vi "Image Acquisition.vi"() -> ()   [LabVIEW 2025]
uses:
  VIs_needed/Grab Manager Mode.ctl
  <vilib>/vision/driver/IMAQdx.llb/IMAQdx Buffer Number Mode.ctl
  <vilib>/Utility/High Resolution Relative Seconds.vi
  <vilib>/vision/driver/NI_Vision_Acquisition_Software.lvlib
  <resource>/objmgr/imaqdx.rc
panel:
  out "Times between Frames":u32
  in  "Output Folder":path
  in  "Stop":bool
  out "Images Saved Per Second":dbl
  out "Images Behind":i32
  out "Images Acquired Per Second":dbl
  in  "Skip Count":u32
  out "Write Speed Waveform":dbl(graph) caption="Image File Write Speed"
  in  "Number of Images":u32=30
  in  "Camera Name":refnum<k21> caption="IMAQdx Session"
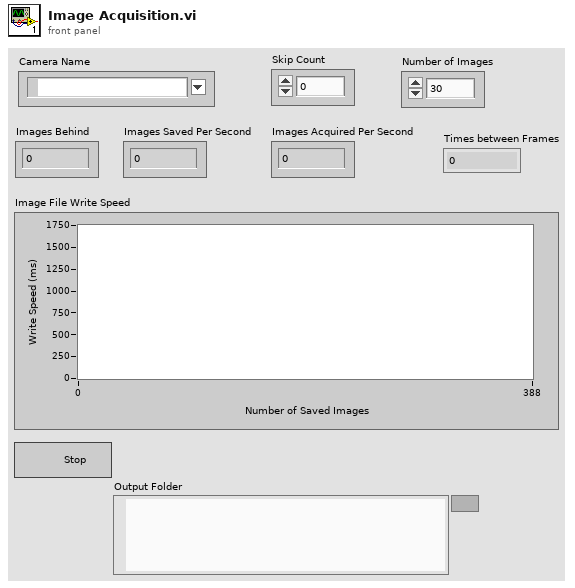
[diagram p1: front panel]
types:
  T1 = typedef "Grab Manager Mode.ctl" = enum16{"Create Processing Images", "Lock", "Add Acquired Image", "Get Acquired Image", "Unlock", "Dispose Processing Images"}
  T2 = cluster{"Number of Processing Images":u32, "Image Border Size":u32}
  T3 = typedef "IMAQdx.ctl" = refnum<k21>
  T4 = typedef "NI_Vision_Acquisition_Software.lvlib/IMAQdx Buffer Number Mode.ctl" = enum32{"Next", "Last", "Buffer Number", "Every", "Last New"}
  T5 = typedef "IMAQ Image.ctl" = refnum<image>
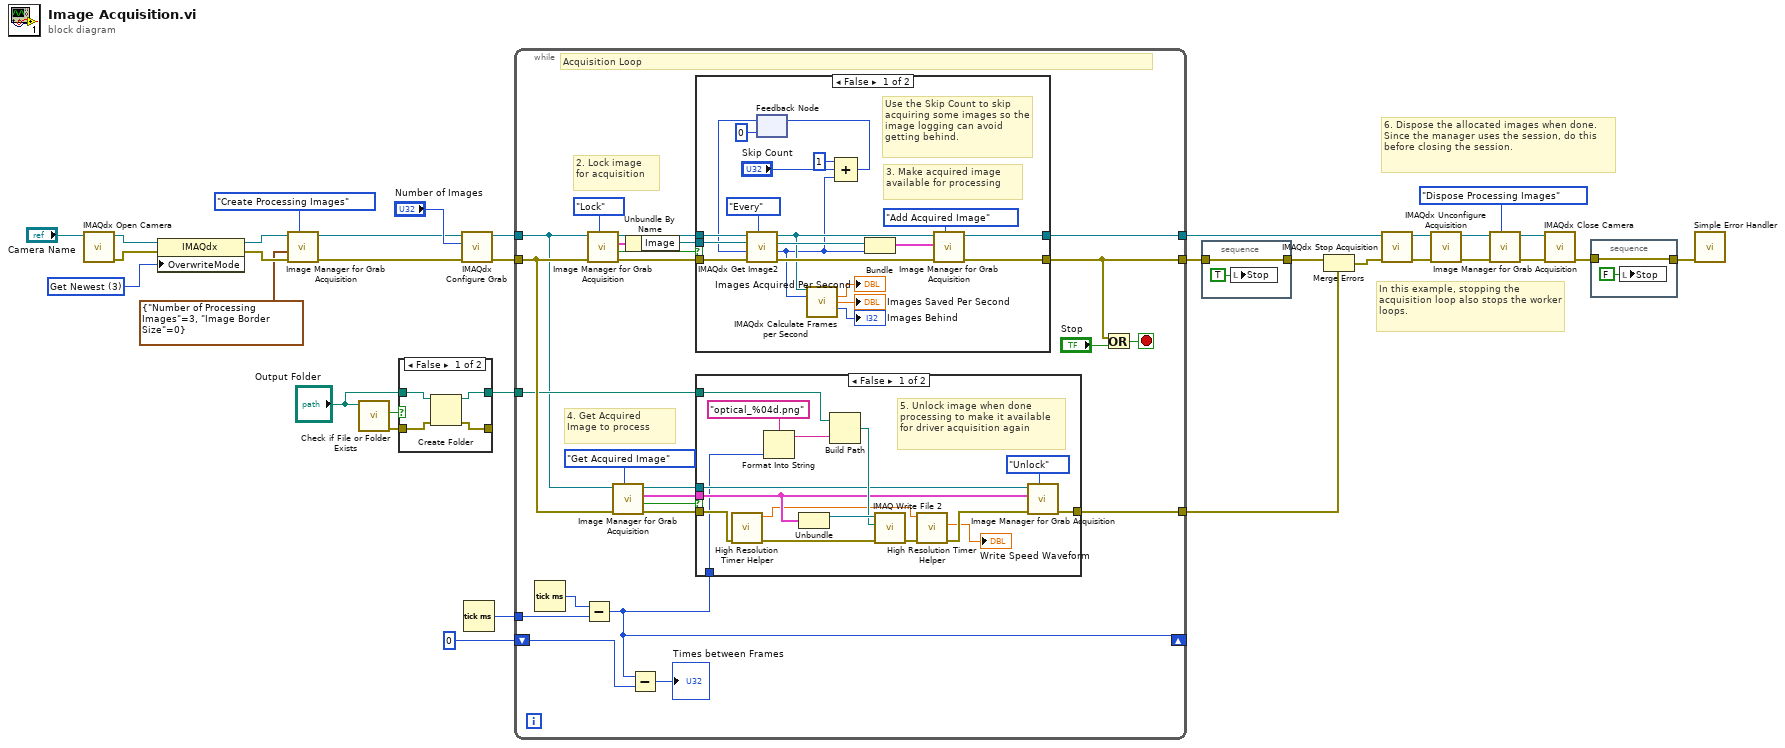
[diagram p0: block diagram]
diagram:
  w32 = u32 3 items=["Get Oldest"=0, "Fail"=2, "Get Newest"=3] ("OverwriteMode")
  # "6. Dispose the allocated images when done. Since the manager uses the session, do this before closing the session."
  # "In this example, stopping the acquisition loop also stops the worker loops."
  n1 = call <vilib>:"IMAQdx Open Camera.vi"("Session In"="Camera Name") -> ("error out"=w28:errorcluster, "Session Out"=w29:T3)  [unwired: 2 in, 7 out]
  n2 = property class="IMAQdx"(reference=w29, error in=w28, "OverwriteMode"=w32) -> (reference out=w31:T3, error out=w30:errorcluster)
  n3 = call "Image Manager for Grab Acquisition.vi"("Mode"=Grab_Manager_Mode."Create Processing Images", "error in (no error)"=w30, "Init Settings"=T2 {"Number of Processing Images"=3, "Image Border Size"=0}, "Session In"=w31) -> ("error out"=w24:errorcluster, "Session Out"=w23:T3)  [unwired: 4 in, 2 out]
  n4 = call <vilib>:"Check if File or Folder Exists.vi"("path"="Output Folder") -> ("error out"=w4:errorcluster, "file or folder exists?"=w6:bool)  [unwired: 8 in, 1 out]
  n5 = case shown="False" w6 {
    tunnel: "Output Folder" -> [w37 w39]
    tunnel: [w36 w39] -> w3
    tunnel: w4 -> [w35 w38]
    tunnel: [w34 w38] -> _
    frame False {
      n6 = Create Folder(path (use dialog)=w37, error in=w35) -> (created path=w36:path, error out=w34:errorcluster)  [unwired: 1 in, 1 out]
    }
    frame True {
    }
  }
  n7 = call <vilib>:"IMAQdx Configure Grab.vi"("error in"=w24, "Number of Buffers"="Number of Images", "Session In"=w23) -> ("error out"=w7:errorcluster, "Session Out"=w8:T3)  [unwired: 7 in]
  n8 = Tick Count (ms)() -> (millisecond timer value=w2:u32)
  n9 = while {
    tunnel: w7 -> [w53]
    tunnel: w8 -> [w51]
    tunnel: [w60] -> w19
    tunnel: [w61] -> w18
    tunnel: w3 -> [w52]
    tunnel: [w50] -> w9
    tunnel: w2 -> [w43]
    shift-right: [w40] -> _
    shift-left: u32 0 -> [w41]
    stop <- w62 stop-if-true
    # "4. Get Acquired Image to process"
    # "2. Lock image for acquisition"
    # "Acquisition Loop"
    n10 = Tick Count (ms)() -> (millisecond timer value=w44:u32)
    n11 = Subtract(x=w44, y=w43) -> (x-y=w40:u32)
    n12 = call "Image Manager for Grab Acquisition.vi"("Mode"=Grab_Manager_Mode."Lock", "error in (no error)"=w53, "Session In"=w51) -> ("error out"=w56:errorcluster, "No Available Image"=w57:bool, "Image Settings Out"=w55:cluster{"Image":T5, "Buffer Number":u32}, "Session Out"=w58:T3)  [unwired: 5 in]
    n13 = call "Image Manager for Grab Acquisition.vi"("Mode"=Grab_Manager_Mode."Get Acquired Image", "error in (no error)"=w53, "Session In"=w51) -> ("error out"=w46:errorcluster, "No Available Image"=w48:bool, "Image Settings Out"=w47:cluster{"Image":T5, "Buffer Number":u32}, "Session Out"=w45:T3)  [unwired: 5 in]
    n14 = Unbundle By Name(w55) -> ("Image"=w54:T5)
    n15 = Subtract(x=w40, y=w41) -> (x-y=→"Times between Frames":u32)
    n16 = case shown="False" w57 {
      tunnel: [w92 w102] -> w60
      tunnel: [w91 w101] -> w61
      tunnel: w58 -> [w100 w102]
      tunnel: w56 -> [w99 w101]
      tunnel: w54 -> [w93 _]
      frame False {
        # "3. Make acquired image available for processing"
        # "Use the Skip Count to skip acquiring some images so the image logging can avoid getting behind."
        n17 = feedback #1(u32 0) -> (w82:u32)
        n18 = call <vilib>:"IMAQdx Get Image2.vi"("Buffer Number Mode (Next)"=IMAQdx_Buffer_Number_Mode."Every", "error in"=w99, "Buffer Number In"=w82, "Image In"=w93, "Session In"=w100) -> ("error out"=w95:errorcluster, "Buffer Number Out"=w86:u32, "Image Out"=w97:T5, "Session Out"=w90:T3)  [unwired: 3 in]
        n19 = call <vilib>:"IMAQdx Calculate Frames per Second.vi"("Session In"=w90, "Buffer Number"=w86) -> ("Acquired Frames per Second"=→"Images Acquired Per Second":dbl, "Processed Frames per Second"=→"Images Saved Per Second":dbl, "Images Behind"=→"Images Behind":i32)  [unwired: 7 in, 4 out]
        n20 = Compound Arithmetic op=ADD(u32 1 ("value"), "Skip Count", w86) -> (w83:u32)
        n21 = feedback-in #1(w83) -> ()
        n22 = Bundle("Image Out"=w97, "Buffer Number Out"=w86) -> (w96:cluster{"Image Out":T5, "Buffer Number Out":u32})  [unwired: 1 in]
        n23 = call "Image Manager for Grab Acquisition.vi"("Mode"=Grab_Manager_Mode."Add Acquired Image", "error in (no error)"=w95, "Image Settings In"=w96, "Session In"=w90) -> ("error out"=w91:errorcluster, "Session Out"=w92:T3)  [unwired: 4 in, 2 out]
      }
      frame True {
        # "The Lock function already has a delay inside when no images are available to prevent loop from going too fast and starving the worker threads from getting processing time."
        # "Write to disk operation is taking longer so images aren't added back to manager. Wait until there is an available image"
      }
    }
    n24 = case shown="False" w48 {
      tunnel: w46 -> [w70 w80]
      tunnel: w47 -> [w72 _]
      tunnel: [w74 w80] -> w50
      tunnel: w52 -> [w78 _]
      tunnel: w45 -> [w71 _]
      tunnel: w40 -> [w64 _]
      frame False {
        # "5. Unlock image when done processing to make it available for driver acquisition again"
        n25 = call "High Resolution Timer Helper.vi"("error in (no error)"=w70) -> ("error out"=w69:errorcluster, "Current Time"=w65:dbl)  [unwired: 8 in, 1 out]
        n26 = Format Into String(format string="optical_%04d.png", w64) -> (resulting string=w77:string)  [unwired: 2 in, 1 out]
        n27 = Unbundle(w72) -> ("Image"=w79:T5)  [unwired: 1 out]
        n28 = Build Path(base path=w78, name or relative path=w77) -> (appended path=w75:path)
        n29 = call-poly "IMAQ Write File 2"("error in (no error)"=w69, "File Path"=w75, "Image"=w79) -> ("error out"=w68:errorcluster)  [unwired: 7 in, 1 out]
        n30 = call "High Resolution Timer Helper.vi"("error in (no error)"=w68, "Previous Time"=w65) -> ("error out"=w67:errorcluster, "Time Difference (ms)"=→"Write Speed Waveform":dbl)  [unwired: 7 in, 1 out]
        n31 = call "Image Manager for Grab Acquisition.vi"("Mode"=Grab_Manager_Mode."Unlock", "error in (no error)"=w67, "Image Settings In"=w72, "Session In"=w71) -> ("error out"=w74:errorcluster)  [unwired: 4 in, 3 out]
      }
      frame True {
        # "No acquired images to process"
      }
    }
    n32 = Or(x=w61, y="Stop") -> (x .or. y?=w62:bool)
  }
  n33 = stacked-sequence {
    tunnel: [w103] -> w17
    tunnel: w18 -> [w103]
    frame #0 {
      n34 = local write "Stop"(TRUE ("Stop")) -> ()
    }
  }
  n35 = Merge Errors(w17, w9) -> (w20:errorcluster)
  n36 = call <vilib>:"IMAQdx Stop Acquisition.vi"("error in"=w20, "Session In"=w19) -> ("error out"=w21:errorcluster, "Session Out"=w22:T3)  [unwired: 8 out]
  n37 = call <vilib>:"IMAQdx Unconfigure Acquisition.vi"("error in"=w21, "Session In"=w22) -> ("error out"=w14:errorcluster, "Session Out"=w15:T3)  [unwired: 8 out]
  n38 = call "Image Manager for Grab Acquisition.vi"("Mode"=Grab_Manager_Mode."Dispose Processing Images", "error in (no error)"=w14, "Session In"=w15) -> ("error out"=w11:errorcluster, "Session Out"=w12:T3)  [unwired: 5 in, 2 out]
  n39 = call <vilib>:"IMAQdx Close Camera.vi"("error in"=w11, "Session In"=w12) -> ("error out"=w10:errorcluster)  [unwired: 9 out]
  n40 = stacked-sequence {
    tunnel: [w105] -> w16
    tunnel: w10 -> [w105]
    frame #0 {
      n41 = local write "Stop"(FALSE ("Stop")) -> ()
    }
  }
  n42 = call <vilib>:"Simple Error Handler.vi"("error in (no error)"=w16) -> ()  [unwired: 4 in, 5 out]
